vi "ChamberModel.vi"(7 "Enable Temperature Control":bool, 10 "Shock Setpoint":dbl format="%#_13g", 11 "Temperature Setpoint":dbl format="%#_13g") -> (2 "Shock Feedback":dbl format="%#_13g", 3 "Temperature Feedback":dbl=75.0 format="%#_13g")   [LabVIEW 2026]
uses:
  <vilib>/Analysis/baseanly.llb/Mean (DBL).vi
  <vilib>/numeric/Random Number (Range) DBL.vi
  <vilib>/Analysis/NI_AALBase.lvlib
  <vilib>/ptbypt/NI_PtbyPt.lvlib
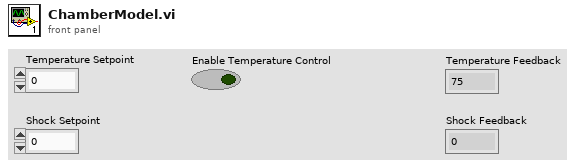
[diagram p1: front panel]
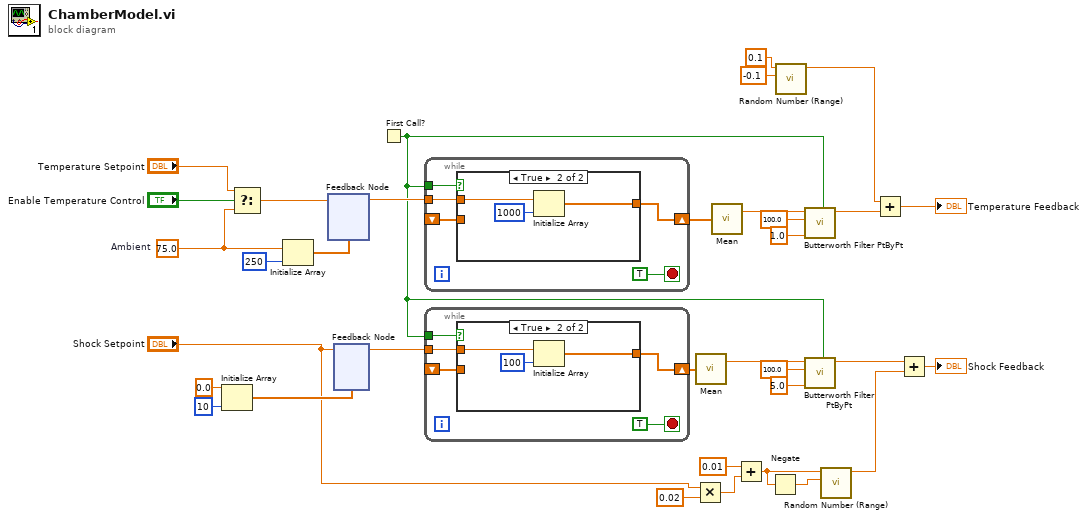
[diagram p0: block diagram]
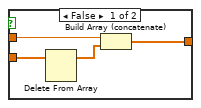
[diagram p2: hidden frame]
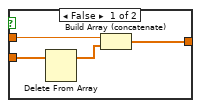
[diagram p3: hidden frame]
diagram:
  w32 = 75.0  # Ambient
  n1 = Initialize Array(0.0 ("element"), 10 ("dimension size")) -> (w28:dbl[])
  n2 = Select(t="Temperature Setpoint", s="Enable Temperature Control", f=w32) -> (s? t:f=w15:dbl)
  n3 = Initialize Array(w32, 250 ("dimension size")) -> (w30:dbl[])
  n4 = feedback #1(w30) -> (w25:dbl)
  n5 = feedback-in #1(w15) -> ()
  n6 = feedback #2(w28) -> (w23:dbl)
  n7 = feedback-in #2("Shock Setpoint") -> ()
  n8 = First Call?() -> (First Call?: T/F=w14:bool)
  n9 = while {
    tunnel: w25 -> [w39]
    tunnel: w14 -> [w38]
    shift-right: [w37] -> w26
    shift-left: _ -> [w36]
    stop <- TRUE stop-if-true
    n10 = case shown="True" w38 {
      tunnel: w39 -> [w42 w46]
      tunnel: [w40 w44] -> w37
      tunnel: w36 -> [w43 _]
      frame False {
        n11 = Delete From Array(array=w43) -> (array with subset deleted=w41:dbl[])  [unwired: 2 in, 1 out]
        n12 = Build Array (concatenate)(w42, w41) -> (w40:dbl[])
      }
      frame True {
        n13 = Initialize Array(w46, 1000 ("dimension size")) -> (w44:dbl[])
      }
    }
  }
  n14 = while {
    tunnel: w23 -> [w51]
    tunnel: w14 -> [w50]
    shift-right: [w49] -> w24
    shift-left: _ -> [w48]
    stop <- TRUE stop-if-true
    n15 = case shown="True" w50 {
      tunnel: w51 -> [w54 w58]
      tunnel: [w52 w56] -> w49
      tunnel: w48 -> [w55 _]
      frame False {
        n16 = Delete From Array(array=w55) -> (array with subset deleted=w53:dbl[])  [unwired: 2 in, 1 out]
        n17 = Build Array (concatenate)(w54, w53) -> (w52:dbl[])
      }
      frame True {
        n18 = Initialize Array(w58, 100 ("dimension size")) -> (w56:dbl[])
      }
    }
  }
  n19 = Multiply(x="Shock Setpoint", y=0.02) -> (x*y=w10:dbl)
  n20 = call-poly <vilib>:"Mean.vi"("X"=w24) -> ("mean"=w22:dbl)  [unwired: 1 out]
  n21 = call-poly <vilib>:"Mean.vi"("X"=w26) -> ("mean"=w21:dbl)  [unwired: 1 out]
  n22 = Add(x=0.01, y=w10) -> (x+y=w7:dbl)
  n23 = Negate(x=w7) -> (-x=w11:dbl)
  n24 = call-poly <vilib>:"Random Number (Range).vi"("lower bound (0)"=-0.1, "upper bound (100)"=0.1) -> ("number"=w13:dbl)  [unwired: 9 in]
  n25 = call <vilib>:"Butterworth Filter PtByPt.vi"("initialize"=w14, "low cutoff freq: fl"=1.0, "sampling freq: fs"=100.0, "x"=w21) -> ("Filtered x"=w20:dbl)  [unwired: 5 in, 1 out]
  n26 = call <vilib>:"Butterworth Filter PtByPt.vi"("initialize"=w14, "low cutoff freq: fl"=5.0, "sampling freq: fs"=100.0, "x"=w22) -> ("Filtered x"=w8:dbl)  [unwired: 5 in, 1 out]
  n27 = call-poly <vilib>:"Random Number (Range).vi"("lower bound (0)"=w11, "upper bound (100)"=w7) -> ("number"=w9:dbl)  [unwired: 9 in]
  n28 = Add(x=w13, y=w20) -> (x+y=→"Temperature Feedback":dbl)
  n29 = Add(x=w8, y=w9) -> (x+y=→"Shock Feedback":dbl)
